vi "Cluster to Element Details.vi"(8 "error in":errorcluster, 11 "cluster":variant) -> (0 "error out":errorcluster, 1 "enum metadata":T1[](array[typedef]), 2 "nested message clusters":variant[](array[variant]), 3 "message metadata":T2)   [LabVIEW 2019, in "grpc-lvsupport.lvlib"]
uses:
  grpc-lvsupport.lvlib
  typeDefs/Message Metadata.ctl
  typeDefs/Message Element Metadata.ctl
  typeDefs/Message Element Type.ctl
  typeDefs/Enum Metadata.ctl
  <vilib>/Utility/Data Type/NI_Data Type.lvlib
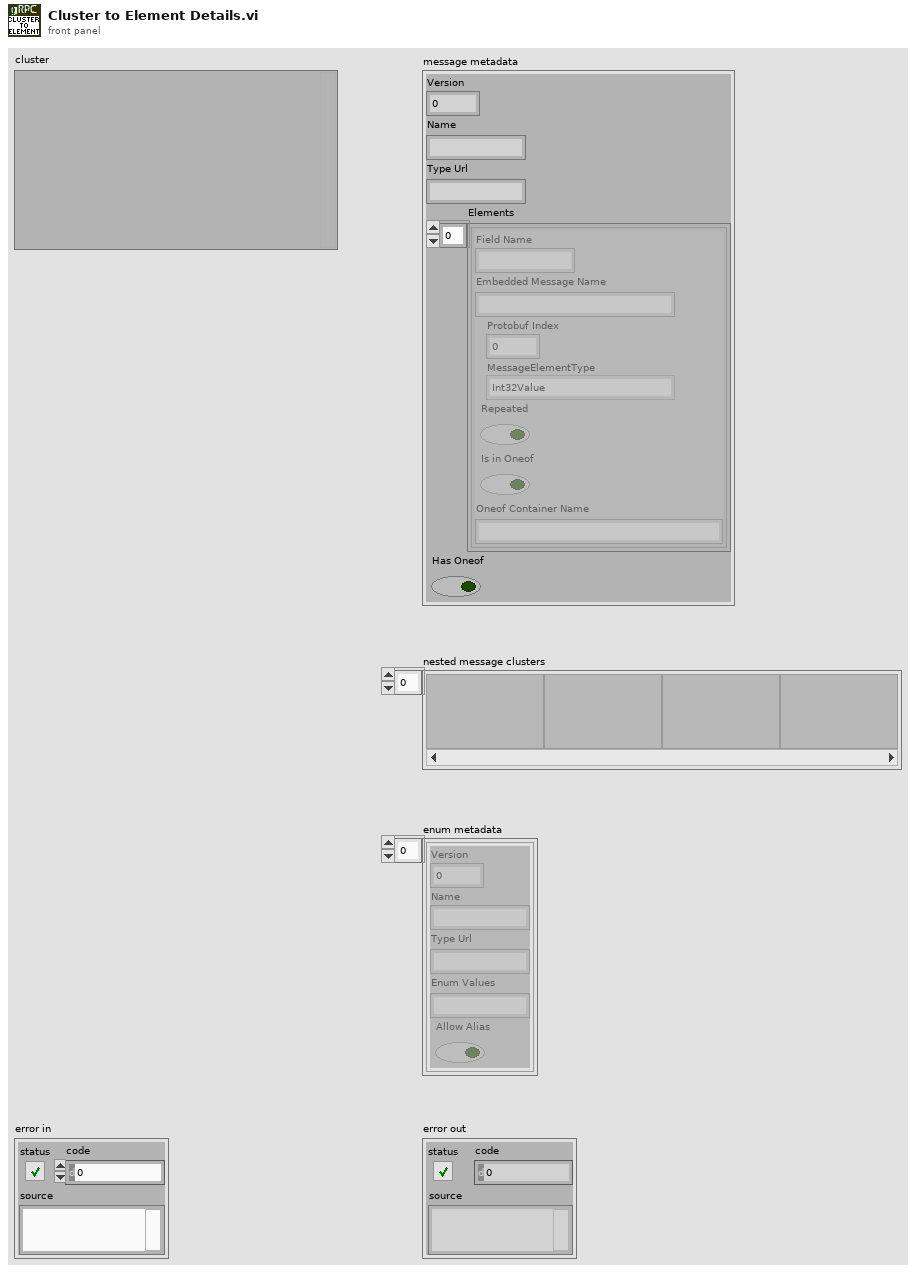
[diagram p1: front panel]
types:
  T1 = typedef "grpc-lvsupport.lvlib/Enum Metadata.ctl" = cluster{"Version":i32, "Name":string, "Type Url":string, "Enum Values":string, "Allow Alias":bool}
  T2 = typedef "grpc-lvsupport.lvlib/Message Metadata.ctl" = cluster{"Version":i32, "Name":string, "Type Url":string, "Elements":T3[], "Has Oneof":bool}
  T3 = typedef "grpc-lvsupport.lvlib/Message Element Metadata.ctl" = cluster{"Field Name":string, "Embedded Message Name":string, "Protobuf Index":i32, "MessageElementType":T4, "Repeated":bool, "Is in Oneof":bool, "Oneof Container Name":string}
  T4 = typedef "grpc-lvsupport.lvlib/Message Element Type.ctl" = enum32{"Int32Value", "FloatValue", "DoubleValue", "BoolValue", "StringValue", "MessageValue", "Int64Value", "UInt32Value", "UInt64Value", "EnumValue", "Bytes", "Fixed64", "Fixed32", "SFixed64", "SFixed32", "SInt64", "SInt32"}
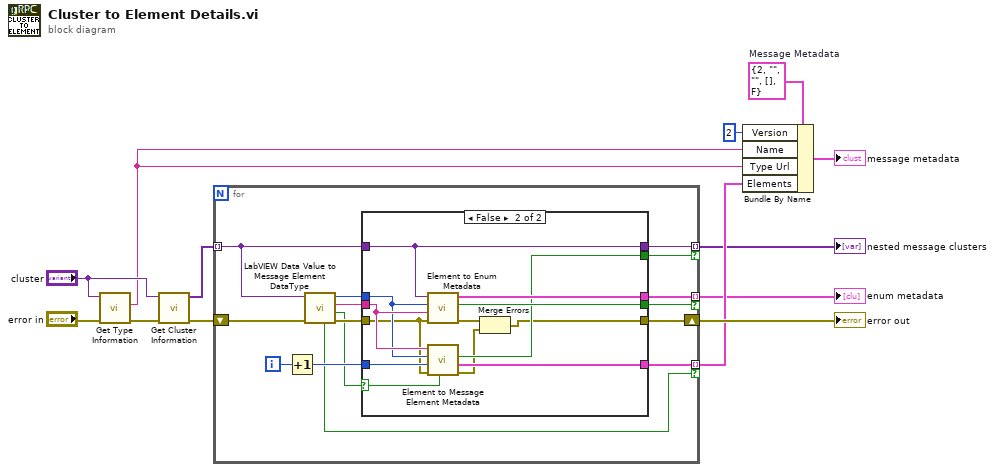
[diagram p0: block diagram]
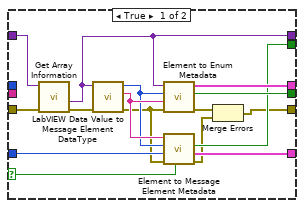
[diagram p2: hidden frame]
diagram:
  w9 = T2 {"Version"=2, "Name"="", "Type Url"="", "Elements"=[], "Has Oneof"=FALSE}  # Message Metadata
  n1 = call <vilib>:"Get Type Information.vi"("error in (no error)"="error in", "variant"="cluster") -> ("error out"=w13:errorcluster, "name"=w5:string)  [unwired: 5 in, 3 out]
  n2 = call <vilib>:"Get Cluster Information.vi"("error in (no error)"=w13, "variant"="cluster") -> ("error out"=w12:errorcluster, "cluster elements"=w6:variant[])  [unwired: 8 in]
  n3 = for {
    tunnel: w6 -> [w17] mode=indexing
    tunnel: [w25] -> w4 mode=indexing if=w16
    shift-right: [w27] -> w11
    shift-left: w12 -> [w18]
    tunnel: [w23] -> w3 mode=indexing if=w22
    tunnel: [w20] -> w1 mode=indexing if=w19
    i -> [w26]
    n4 = Increment(x=w26) -> (x+1=w24:i32)
    n5 = call "LabVIEW Data Value to Message Element DataType.vi"("error in"=w18, "message value"=w17) -> ("error out"=w28:errorcluster, "array"=w15:bool, "message name"=w14:string, "message element type"=w21:T4, "supported"=w16:bool)  [unwired: 5 in]
    n6 = case shown="False" w15 {
      selector: w15 -> [w34 w50]
      tunnel: w24 -> [w35 w51]
      tunnel: [w32 w49] -> w25
      tunnel: w28 -> [w44 w48]
      tunnel: w17 -> [w43 w57]
      tunnel: [w30 w45] -> w27
      tunnel: [w39 w57] -> w23
      tunnel: [w33 w54] -> w22
      tunnel: w21 -> [_ w52]
      tunnel: [w40 w56] -> w20
      tunnel: [w41 w55] -> w19
      tunnel: w14 -> [_ w53]
      frame True {
        n7 = call <vilib>:"Get Array Information.vi"("error in (no error)"=w44, "variant"=w43) -> ("error out"=w38:errorcluster, "array element data type"=w39:variant)  [unwired: 6 in, 2 out]
        n8 = call "LabVIEW Data Value to Message Element DataType.vi"("error in"=w38, "message value"=w39) -> ("error out"=w31:errorcluster, "message name"=w37:string, "message element type"=w36:T4)  [unwired: 5 in, 2 out]
        n9 = call "Element to Enum Metadata.vi"("error in (no error)"=w31, "Name"=w37, "MessageElementType"=w36, "Element"=w39) -> ("error out"=w42:errorcluster, "Is Enum?"=w41:bool, "Enum Metadata"=w40:T1)  [unwired: 5 in]
        n10 = call "Element to Message Element Metadata.vi"("repeated"=w34, "error in"=w31, "protobuf index"=w35, "message element type"=w36, "message name"=w37) -> ("error out"=w29:errorcluster, "element metadata"=w32:T3, "nested cluster"=w33:bool)  [unwired: 4 in]
        n11 = Merge Errors(w42, w29) -> (w30:errorcluster)
      }
      frame False {
        n12 = call "Element to Enum Metadata.vi"("error in (no error)"=w48, "Name"=w53, "MessageElementType"=w52, "Element"=w57) -> ("error out"=w47:errorcluster, "Is Enum?"=w55:bool, "Enum Metadata"=w56:T1)  [unwired: 5 in]
        n13 = call "Element to Message Element Metadata.vi"("repeated"=w50, "error in"=w48, "protobuf index"=w51, "message element type"=w52, "message name"=w53) -> ("error out"=w46:errorcluster, "element metadata"=w49:T3, "nested cluster"=w54:bool)  [unwired: 4 in]
        n14 = Merge Errors(w47, w46) -> (w45:errorcluster)
      }
    }
  }
  "nested message clusters" <- w3
  "error out" <- w11
  "enum metadata" <- w1
  n15 = Bundle By Name(cluster=w9, "Version"=2, "Name"=w5, "Type Url"=w5, "Elements"=w4) -> (→"message metadata":T2)
